vi "CSE routine - Script Instance Manager.vi"(4 "Close if topmost only (f)":bool, 6 "cmd (open)":enum16{"open", "close inst", "close all"}(ring), 8 "error in":errorcluster, 10 "Script Name":string, 11 "Caller CSE RefNum":T1) -> (0 "error out":errorcluster, 1 "Error message":string, 3 "new CSE RefNum":T1)   [LabVIEW 2021]
doc: "::: CalcExpress Toolkit :::\nCopyright (c) 2000-2026 Konstantin Shifershteyn. All rights reserved."
uses:
  CSE Instance RefNum.ctl
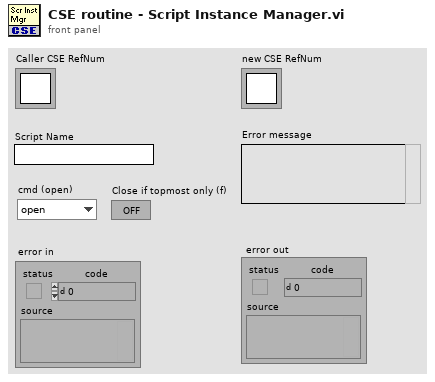
[diagram p1: front panel]
types:
  T1 = typedef "CSE Instance RefNum.ctl" = refnum<k1>
  T2 = cluster{"script path":path, "dup CSE RefNum":T1, string, "error IO":errorcluster}[]
  T3 = cluster{"Topmost Instance Refnum":u32, "Current Instance Level":i32, "Script Name":string}[]
  T4 = cluster{"Topmost Instance Refnum":u32, "Current Instance Level":i32, "Script Name":string}
  T5 = cluster{"script path":path, "dup CSE RefNum":T1, string, "error IO":errorcluster}
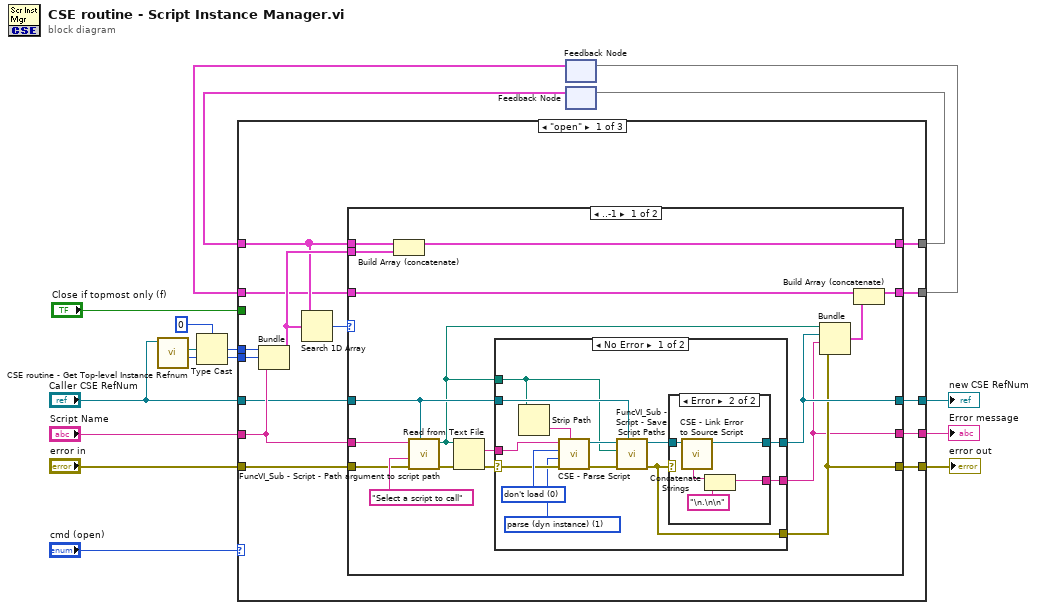
[diagram p0: block diagram]
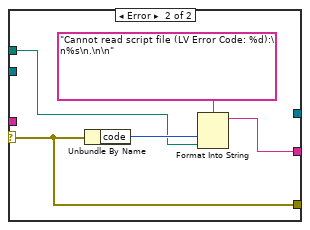
[diagram p3: hidden frame]
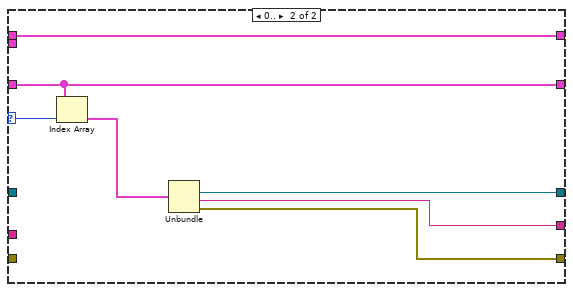
[diagram p4: hidden frame]
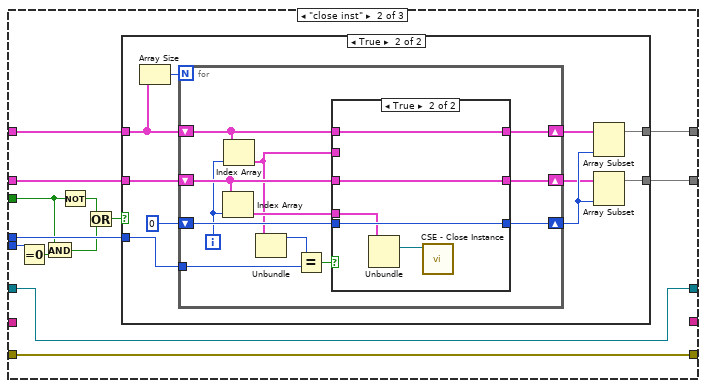
[diagram p5: hidden frame]
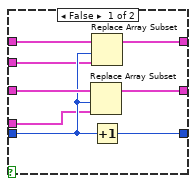
[diagram p7: hidden frame]
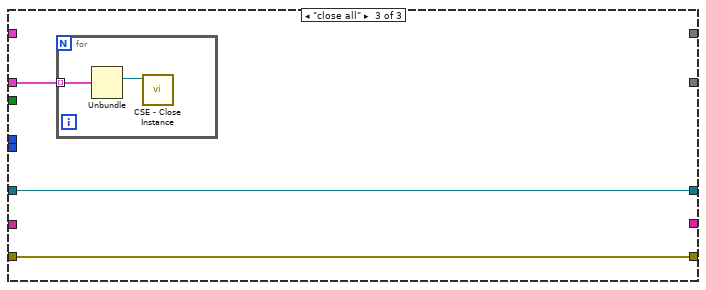
[diagram p8: hidden frame]
diagram:
  n1 = call "CSE routine - Get Top-level Instance Refnum.vi"("CSE Refnum"="Caller CSE RefNum") -> ("Current Instance Level"=w2:i32, "Top-level CSE Instance Refnum"=w8:T1)  [unwired: 7 in, 2 out]
  n2 = Type Cast(type=u32 0 ("Topmost Instance Refnum"), x=w8) -> (*(type *) &x=w11:u32)
  n3 = feedback #1() -> (w3:T2)  [unwired: 1 in]
  n4 = feedback #2() -> (w4:T3)  [unwired: 1 in]
  n5 = case shown="\"open\"" "cmd (open)" {
    tunnel: [w22 w91 w131] -> w16
    tunnel: "error in" -> [w23 w91 w131]
    tunnel: w3 -> [w21 w90 w130]
    tunnel: [w20 w87 _] -> w5
    tunnel: w4 -> [w28 w89 _]
    tunnel: [w30 w88 _] -> w6
    tunnel: "Script Name" -> [w26 _ _]
    tunnel: "Caller CSE RefNum" -> [w25 w85 w129]
    tunnel: w11 -> [w24 w86 _]
    tunnel: [w19 w85 w129] -> w10
    tunnel: [w18 _ _] -> w9
    tunnel: w2 -> [w17 w82 _]
    tunnel: "Close if topmost only (f)" -> [_ w79 _]
    frame "open" {
      n6 = Bundle("Topmost Instance Refnum"=w24, "Current Instance Level"=w17, "Script Name"=w26) -> (w29:T4)  [unwired: 1 in]
      n7 = Search 1D Array(1D array=w28, element=w29) -> (index of element=w27:i32)  [unwired: 1 in]
      n8 = case shown="..-1" w27 {
        selector: w27 -> [_ w77]
        tunnel: [w47 w78] -> w30
        tunnel: w29 -> [w46 _]
        tunnel: w28 -> [w45 w78]
        tunnel: w26 -> [w42 _]
        tunnel: w25 -> [w41 _]
        tunnel: w23 -> [w40 _]
        tunnel: [w33 w72] -> w22
        tunnel: w21 -> [w38 w76]
        tunnel: [w36 w76] -> w20
        tunnel: [w35 w74] -> w19
        tunnel: [w32 w73] -> w18
        frame ..-1 {
          n9 = Build Array (concatenate)(w45, w46) -> (w47:T3)
          n10 = call "FuncVI_Sub - Script - Path argument to script path.vi"("CSE RefNum"=w41, "error in"=w40, "prompt"="Select a script to call", "arg: path"=w42) -> ("error out"=w44:errorcluster, "script path"=w39:path)  [unwired: 6 in]
          n11 = Read from Text File(file (use dialog)=w39, error in=w44) -> (text=w31:string, error out=w34:errorcluster)  [unwired: 2 in, 2 out]
          n12 = case shown="No Error" w34 {
            selector: w34 -> [w54 w69]
            tunnel: w41 -> [w57 _]
            tunnel: w39 -> [w55 w68]
            tunnel: [w52 _] -> w35
            tunnel: [w51 w69] -> w33
            tunnel: [w50 w67] -> w32
            tunnel: w31 -> [w48 _]
            frame No Error {
              w49 = u32 1 items=["parse", "parse (dyn instance)", "test syntax"] ("action")
              w59 = u32 0 items=["don't load", "load", "load & test"] ("load FuncVIs")
              n13 = Strip Path(path=w55) -> (name=w58:string)  [unwired: 1 out]
              n14 = call "CSE - Parse Script.vi"("Script name"=w58, "error in"=w54, "action"=w49, "load FuncVIs"=w59, "Script"=w48) -> ("error out"=w60:errorcluster, "CSE RefNum"=w56:T1)  [unwired: 2 in, 3 out]
              n15 = call "FuncVI_Sub - Script - Save Script Paths.vi"("Caller CSE RefNum"=w57, "error in"=w60, "Script File Path"=w55, "CSE RefNum"=w56) -> ("error out"=w51:errorcluster, "dup CSE RefNum"=w53:T1)  [unwired: 6 in]
              n16 = case shown="Error" w51 {
                tunnel: w53 -> [w61 w66]
                tunnel: [_ w63] -> w50
                tunnel: [w61 w62] -> w52
                frame No Error {
                }
                frame Error {
                  n17 = call "CSE - Link Error to Source Script.vi"("CSE RefNum"=w66) -> ("dup CSE RefNum"=w62:T1, "Error Message"=w65:string)  [unwired: 4 in, 5 out]
                  n18 = Concatenate Strings(w65, "\n.\n\n" ("string")) -> (w63:string)
                }
              }
            }
            frame Error {
              n19 = Unbundle By Name(w69) -> ("code"=w71:i32)
              n20 = Format Into String(format string="Cannot read script file (LV Error Code: %d):\n%s\n.\n\n", w71, w68) -> (resulting string=w67:string)  [unwired: 2 in, 1 out]
            }
          }
          n21 = Bundle("script path"=w39, "dup CSE RefNum"=w35, w32, "error IO"=w33) -> (w37:T5)  [unwired: 1 in]
          n22 = Build Array (concatenate)(w38, w37) -> (w36:T2)
        }
        frame 0.. {
          n23 = Index Array(array=w76, index=w77) -> (element=w75:T5)
          n24 = Unbundle(w75) -> ("dup CSE RefNum"=w74:T1, w73:string, "error IO"=w72:errorcluster)  [unwired: 1 out]
        }
      }
    }
    frame "close inst" {
      n25 = Equal To 0?(x=w82) -> (x = 0?=w81:bool)
      n26 = And(x=w79, y=w81) -> (x .and. y?=w80:bool)
      n27 = Not(x=w79) -> (.not. x?=w84:bool)
      n28 = Or(x=w84, y=w80) -> (x .or. y?=w83:bool)
      n29 = case shown="True" w83 {
        tunnel: w90 -> [w92 w103]
        tunnel: w89 -> [w93 w102]
        tunnel: [w93 w96] -> w88
        tunnel: [w92 w95] -> w87
        tunnel: w86 -> [_ w94]
        frame False {
        }
        frame True {
          n30 = Array Size(array=w102) -> (size(s)=w101:i32)
          n31 = for {
            N: w101 -> [_]
            shift-right: [w111] -> w97
            shift-left: w102 -> [w112]
            shift-right: [w110] -> w98
            shift-left: w103 -> [w107]
            tunnel: w94 -> [w115]
            shift-right: [w108] -> w99
            shift-left: 0 -> [w109]
            i -> [w106]
            n32 = Index Array(array=w107, index=w106) -> (element=w105:T5)
            n33 = Index Array(array=w112, index=w106) -> (element=w104:T4)
            n34 = Unbundle(w104) -> ("Topmost Instance Refnum"=w114:u32)  [unwired: 2 out]
            n35 = Equal?(x=w114, y=w115) -> (x = y?=w113:bool)
            n36 = case shown="True" w113 {
              tunnel: w112 -> [w122 w128]
              tunnel: [w121 w128] -> w111
              tunnel: w107 -> [w123 w126]
              tunnel: [w120 w126] -> w110
              tunnel: w109 -> [w118 w127]
              tunnel: [w119 w127] -> w108
              tunnel: w105 -> [w117 w125]
              tunnel: w104 -> [w116 _]
              frame False {
                n37 = Replace Array Subset(array=w123, new element=w117, index=w118) -> (w120:T2)
                n38 = Replace Array Subset(array=w122, new element=w116, index=w118) -> (w121:T3)
                n39 = Increment(x=w118) -> (x+1=w119:i32)
              }
              frame True {
                n40 = Unbundle(w125) -> ("dup CSE RefNum"=w124:T1)  [unwired: 3 out]
                n41 = call "CSE - Close Instance.vi"("CSE RefNum"=w124) -> ()  [unwired: 6 in, 3 out]
              }
            }
          }
          n42 = Array Subset(array=w97, length=w99) -> (w96:T3)  [unwired: 1 in]
          n43 = Array Subset(array=w98, length=w99) -> (w95:T2)  [unwired: 1 in]
        }
      }
    }
    frame "close all" {
      n44 = for {
        tunnel: w130 -> [w133] mode=indexing
        n45 = Unbundle(w133) -> ("dup CSE RefNum"=w132:T1)  [unwired: 3 out]
        n46 = call "CSE - Close Instance.vi"("CSE RefNum"=w132) -> ()  [unwired: 6 in, 3 out]
      }
    }
  }
  "error out" <- w16
  "new CSE RefNum" <- w10
  "Error message" <- w9
  n47 = feedback-in #1(w5) -> ()
  n48 = feedback-in #2(w6) -> ()
